vi "CSMclient.vi"(7 "CSM Name":string="CSM-Module") -> ()   [LabVIEW 2026, in "UI-距离测量.lvlib" / "UDP.lvlib"]
uses:
  UDP.lvlib
  Supports/UDP Settings.ctl
  Supports/UDP States.ctl
  <userlib>/_NEVSTOP/Communicable State Machine(CSM)/_Polymophic/CSM - Filter Duplicated Lines.vi
  93835eb5-cc1e-40fc-ad4c-6bcb3c5fabc0.vi
  <userlib>/_NEVSTOP/Communicable State Machine(CSM)/_Polymophic/CSM - Replace Marks in Messages.vi
  f33b5746-793c-4b4f-ac6a-ed109ca97768.vi
  <userlib>/_NEVSTOP/Communicable State Machine(CSM)/AdvanceAPI/CSM - Compact Multiple States.vi
  <userlib>/_NEVSTOP/Communicable State Machine(CSM)/AdvanceAPI/CSM - Break Down Multiple States String.vi
  <userlib>/_NEVSTOP/Communicable State Machine(CSM)/_Shared/Remove Comments from Single-line.vi
  <userlib>/_NEVSTOP/Communicable State Machine(CSM)/_Shared/Split Single-line Message.vi
  <userlib>/_NEVSTOP/Communicable State Machine(CSM)/_Shared/Trim Single-line Text.vi
  <userlib>/_NEVSTOP/Communicable State Machine(CSM)/AdvanceAPI/CSM - Revert Arguments-Safe String.vi
  <userlib>/_NEVSTOP/Communicable State Machine(CSM)/AdvanceAPI/CSM - Make String Arguments Safe.vi
  <userlib>/_NEVSTOP/Communicable State Machine(CSM)/AdvanceAPI/CSM - Keywords.vi
  <userlib>/_NEVSTOP/Communicable State Machine(CSM)/addons/API-String-Arugments-Support/_Support/Convert API String Arguments to Data(variant).vi
  <userlib>/_NEVSTOP/Communicable State Machine(CSM)/addons/API-String-Arugments-Support/_Support/Data To API String Arguments.vi
  <userlib>/_NEVSTOP/Communicable State Machine(CSM)/Communicable State Machine.lvlib
  <userlib>/_NEVSTOP/Communicable State Machine(CSM)/addons/Loop-Support/CSM Loop Support.lvlib
panel:
  in  "Start":bool
  in  "停止":bool
  out "data out":string
  out "Error Occurred":errorcluster
  out "State History":string
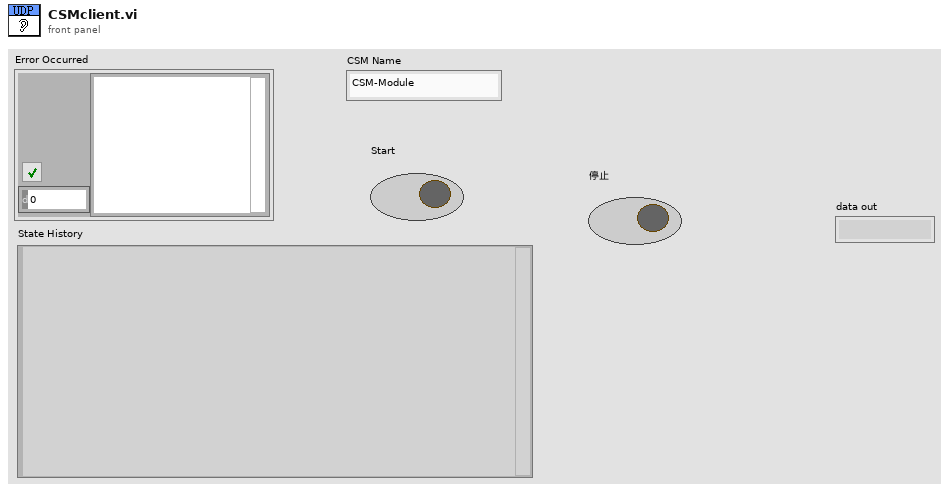
[diagram p1: front panel]
types:
  T1 = typedef "UI-距离测量.lvlib/UDP.lvlib/UDP Settings.ctl" = cluster{"连接ID":refnum<k16>, "网络地址(字符串)":string, "地址":u32, "本端口":u16, "对向":u16, "Read Interval":dbl, "Write Interval":dbl}
  T2 = enum32{"Invalid", "Standard", "Closed", "Hidden", "Minimized", "Maximized"}
  T3 = enum32{"invalid app kind", "Development System", "Run Time System", "Student Edition", "Embedded LabVIEW", "Evaluation", "Custom"}
  T4 = typedef "UI-距离测量.lvlib/UDP.lvlib/UDP States.ctl" = enum16{"Idle", "Acquiring", "Error"}
  T5 = typedef "Communicable State Machine.lvlib/_CSM_Response Source Message.ctl" = cluster{"‘State":string, "’Arguments":string, "’Error":errorcluster}
  T6 = cluster{"Current VI Reference":refnum<vi>, "Close Panel on Exit?":bool}
  T7 = cluster{"Core":cluster{"Current VI Reference":refnum<vi>, "Close Panel on Exit?":bool}, "State":T4, "UDP Settings":T1, "采集时间":timestamp}
  T8 = typedef "全局变量数据.ctl" = cluster{"温度采集":dbl[], "温度控制":dbl[], "压力测量":dbl[], "Zolix":dbl[], "步进电机":dbl[], "湿度测量":dbl[], "距离测量":dbl[]}
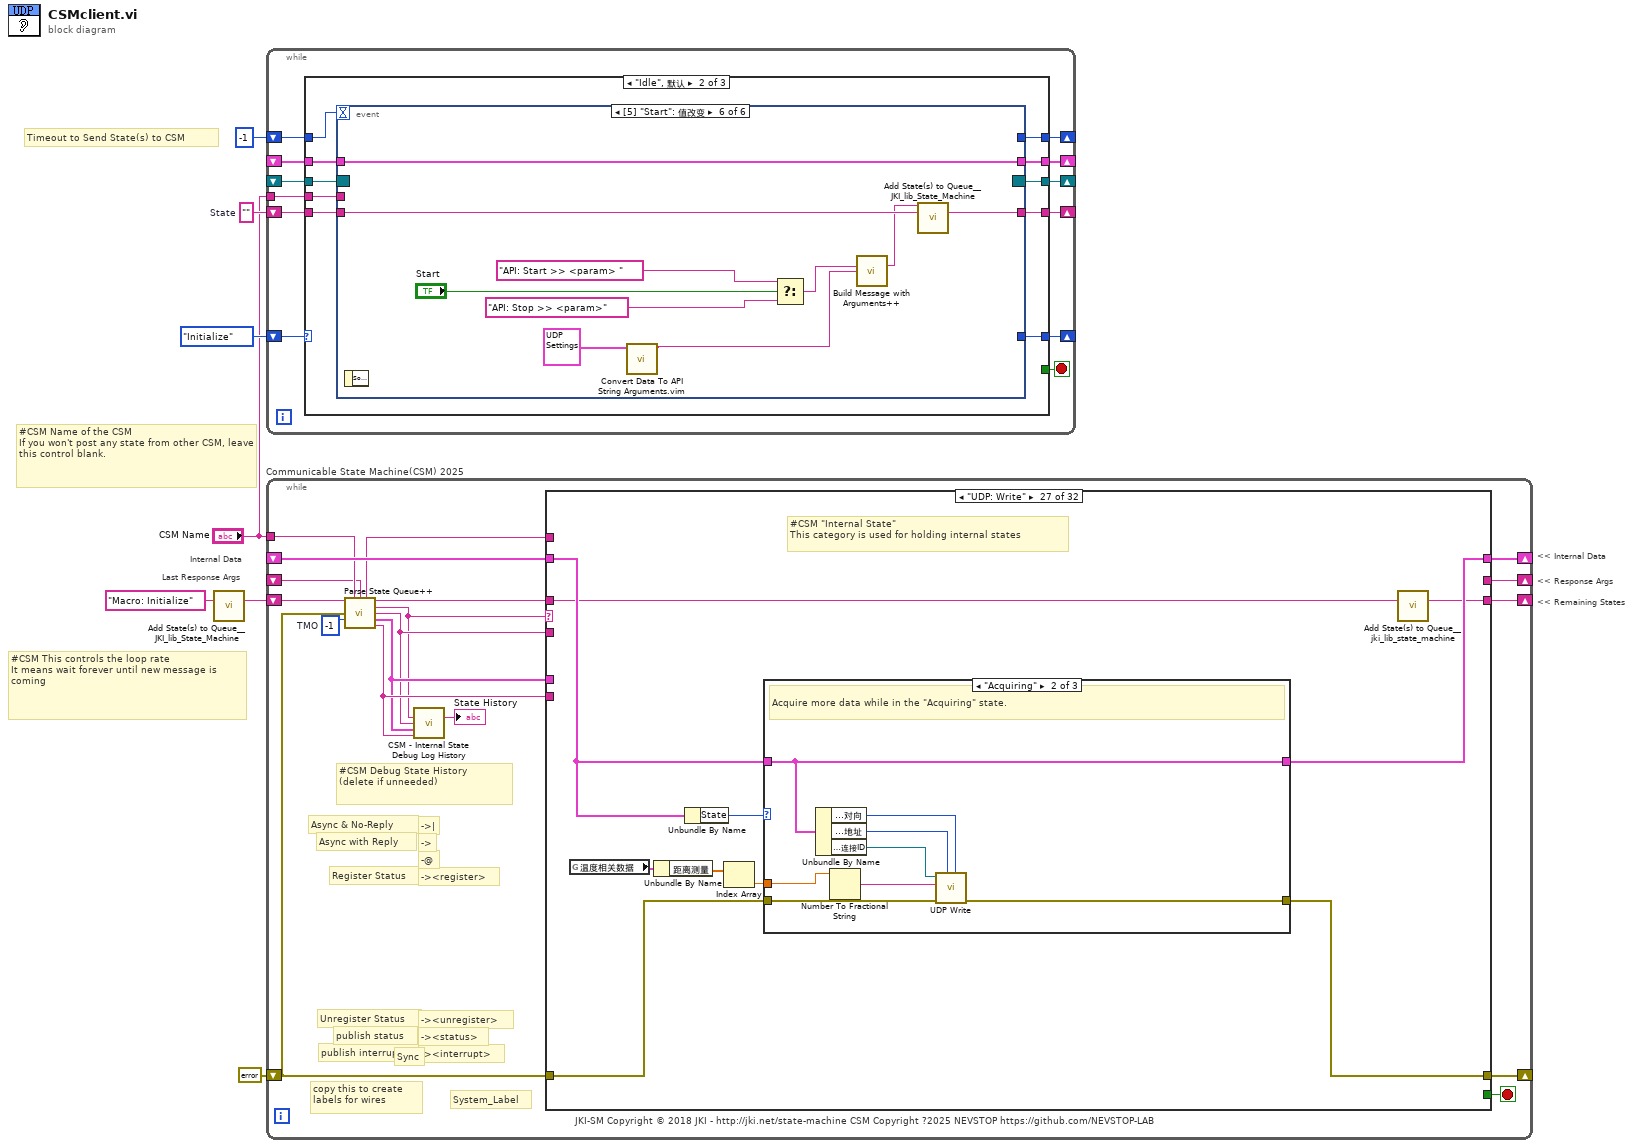
[diagram p0: block diagram]
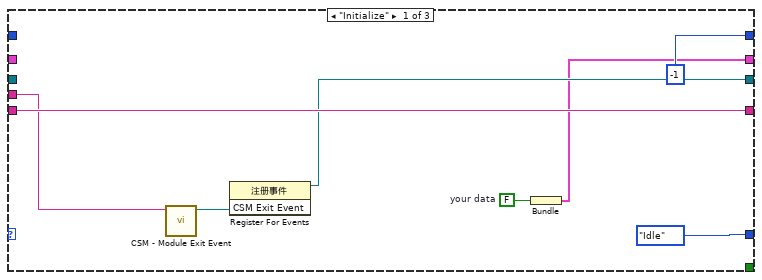
[diagram p2: hidden frame]
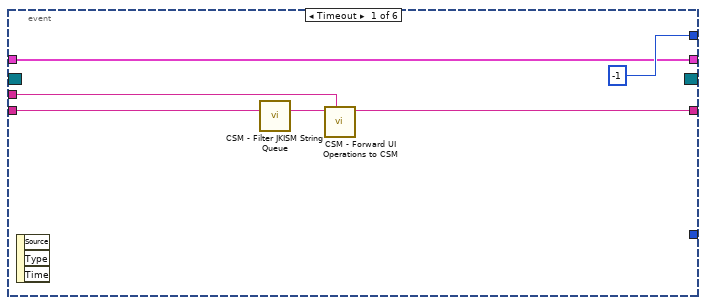
[diagram p3: hidden frame]
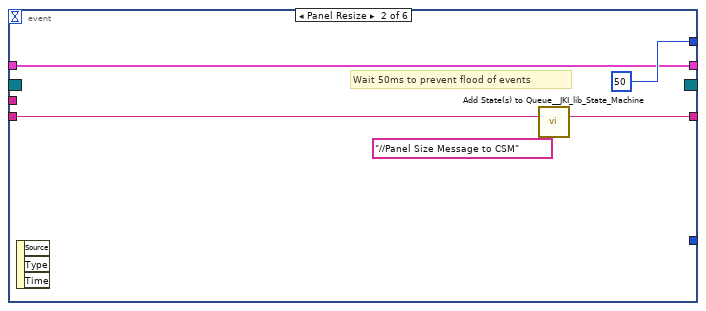
[diagram p4: hidden frame]
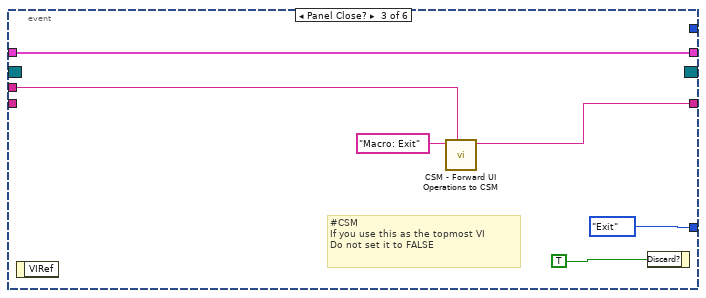
[diagram p5: hidden frame]
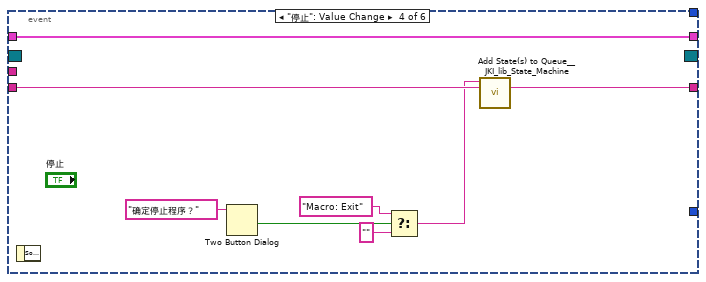
[diagram p6: hidden frame]
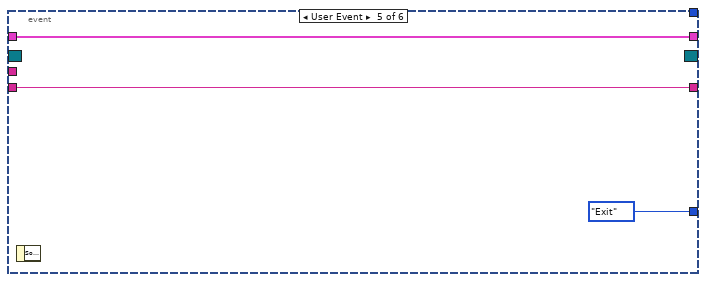
[diagram p7: hidden frame]
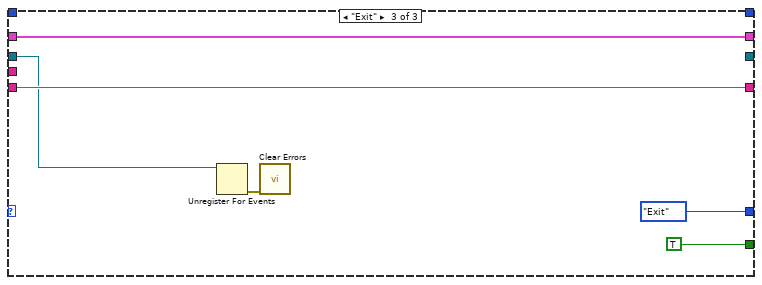
[diagram p8: hidden frame]
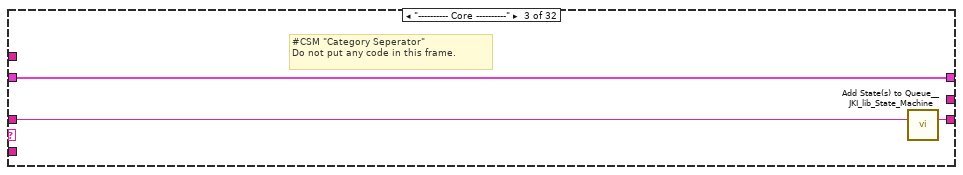
[diagram p11: hidden frame]
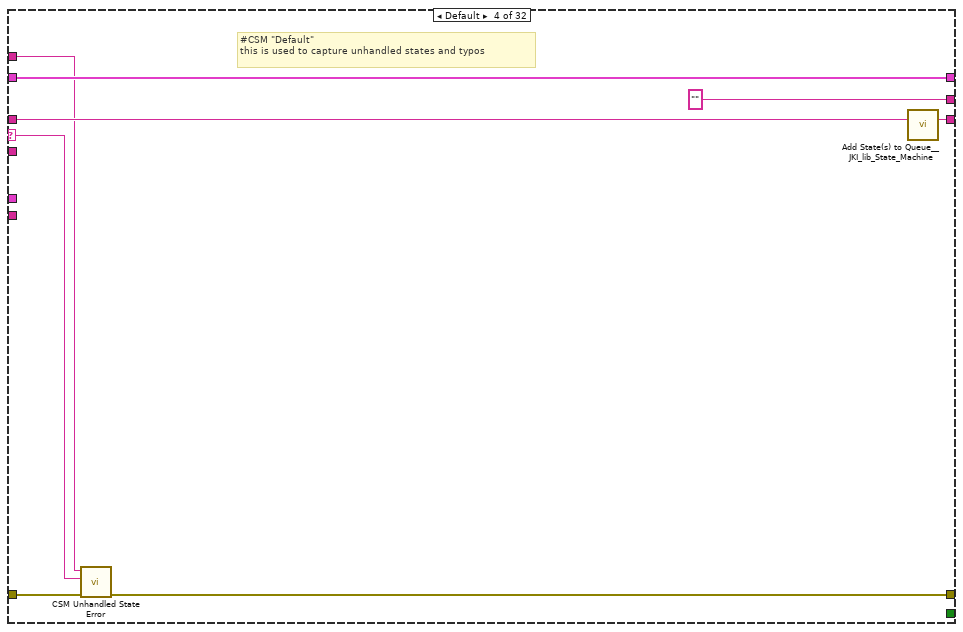
[diagram p12: hidden frame]
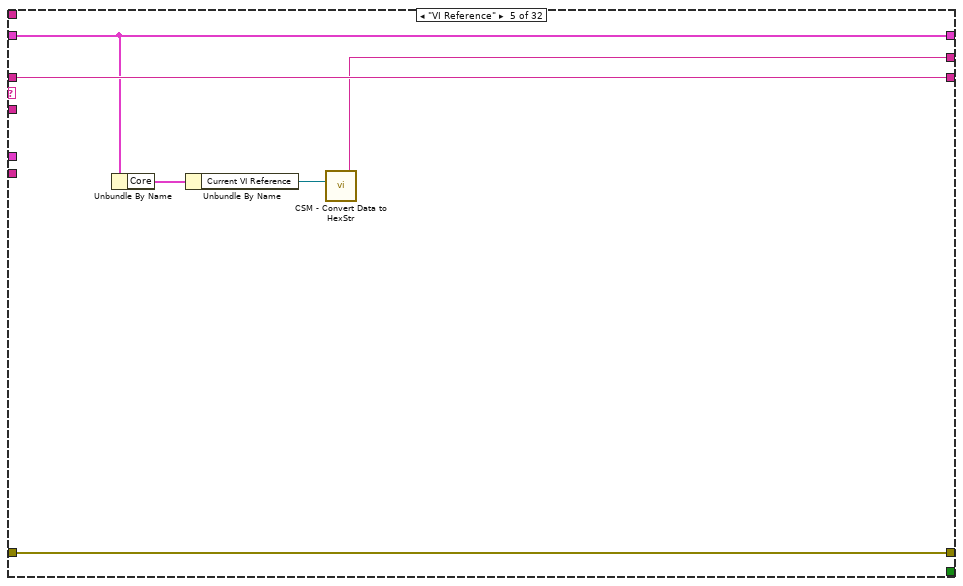
[diagram p13: hidden frame]
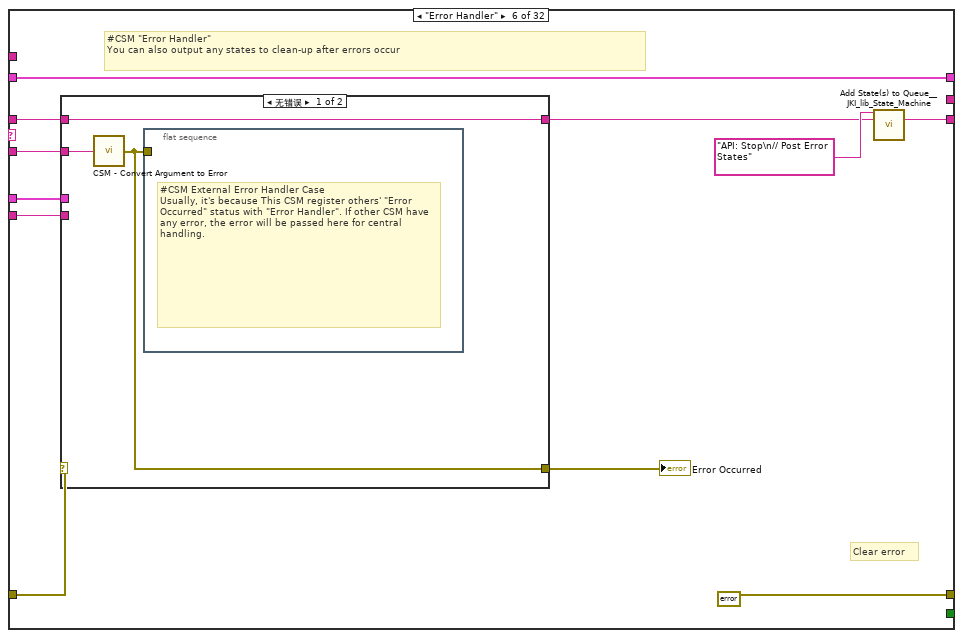
[diagram p14: hidden frame]
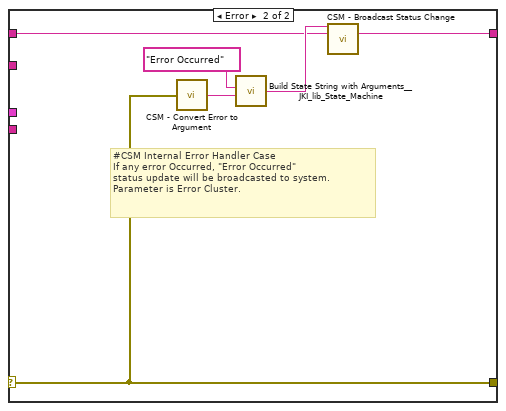
[diagram p15: hidden frame]
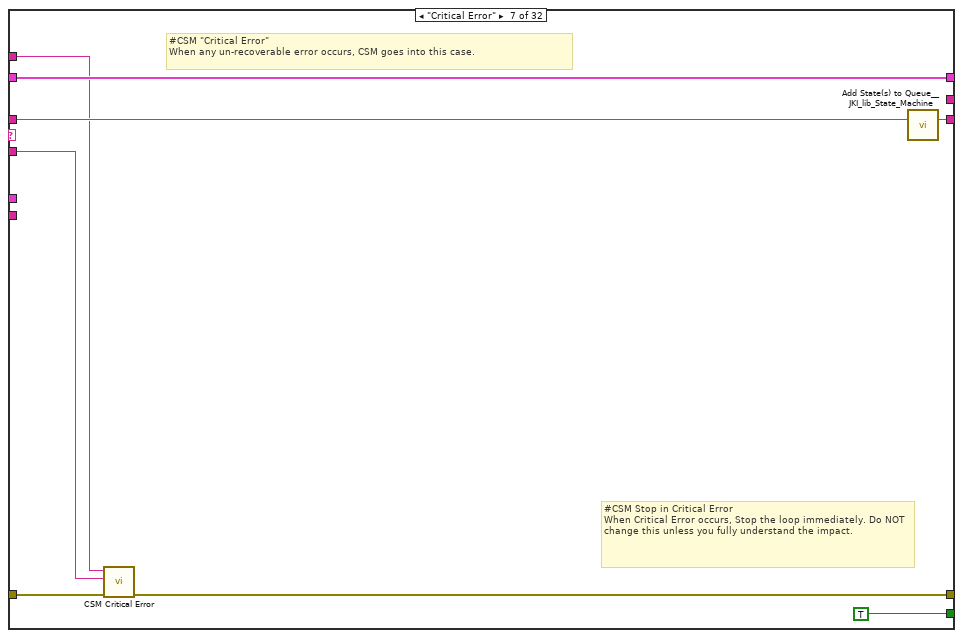
[diagram p16: hidden frame]
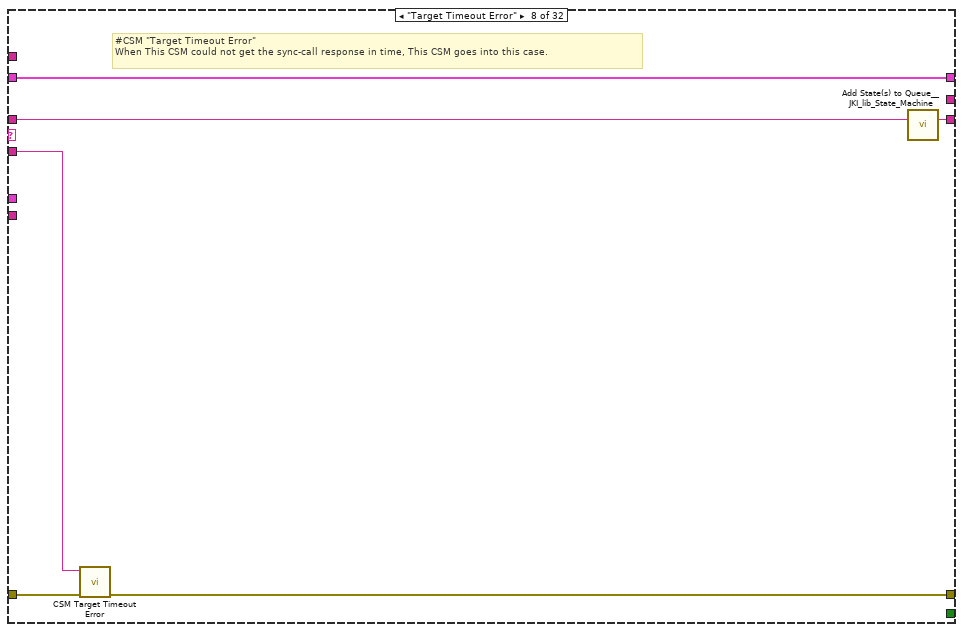
[diagram p17: hidden frame]
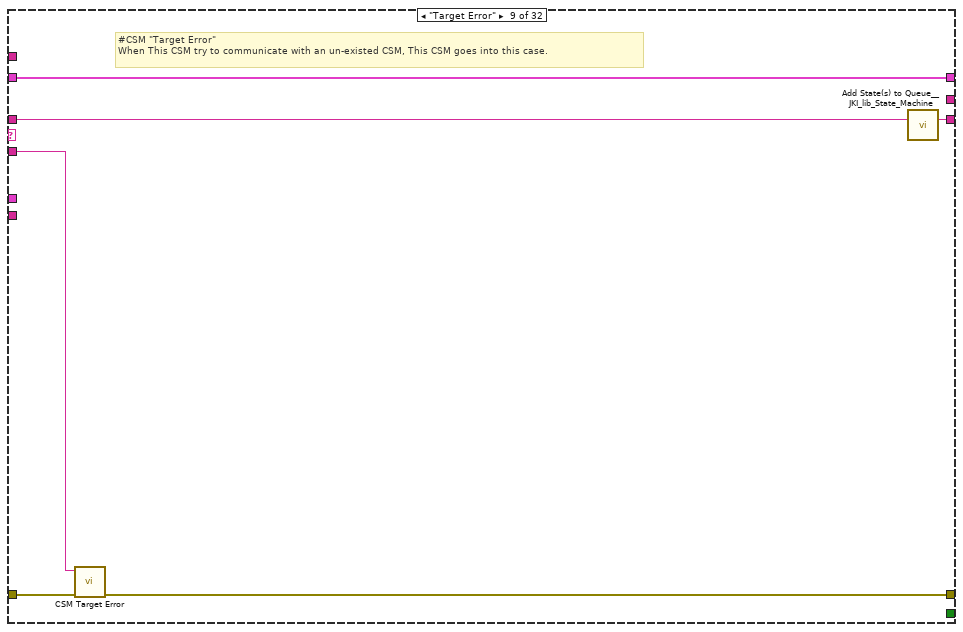
[diagram p18: hidden frame]
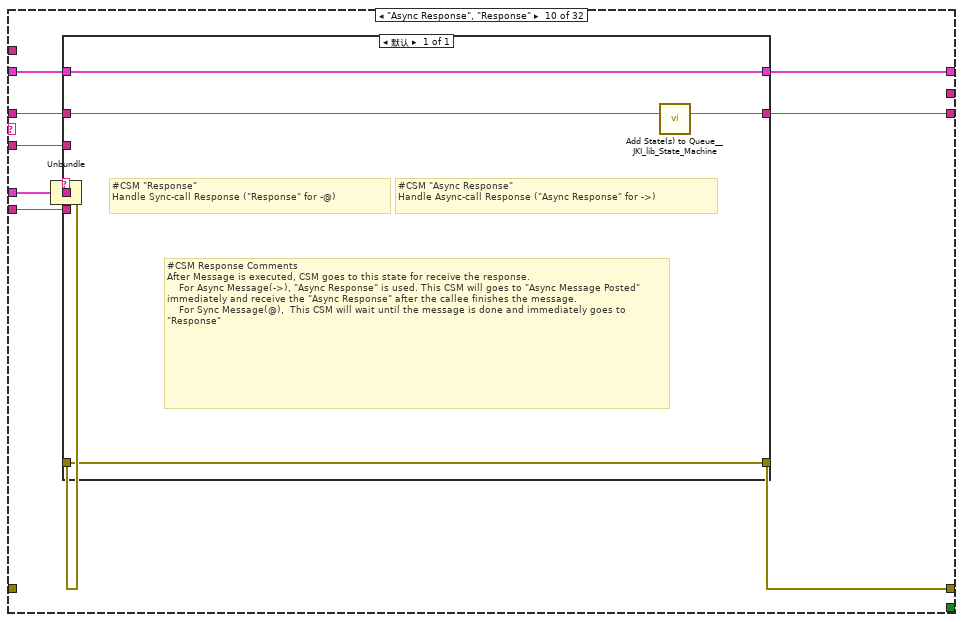
[diagram p19: hidden frame]
diagram:
  w3 = ""  # State
  # "Timeout to Send State(s) to CSM"
  # "Last Response Args"
  # "Internal Data"
  # "#CSM Name of the CSM\nIf you won't post any state from other CSM, leave this control blank."
  # "#CSM This controls the loop rate\nIt means wait forever until new message is coming"
  # "<< Internal Data"
  # "<< Response Args"
  # "<< Remaining States"
  n1 = call <vilib>:"Add State(s) to Queue__JKI_lib_State_Machine.vi"("State(s) in (\"\")"="Macro: Initialize" ("Init State(\"Macro: Initialize\")")) -> ("States Out"=w5:string)  [unwired: 14 in]
  n2 = while {
    shift-right: [w18] -> _
    shift-left: enum16{"Idle", "Initialize", "Exit"}."Initialize" -> [w19]
    tunnel: "CSM Name" -> [w16]
    shift-right: [w14] -> _
    shift-left: w3 -> [w15]
    shift-right: [w12] -> _
    shift-left: -1 -> [w13]
    shift-right: [w11] -> _
    shift-left: _ -> [w10]
    shift-right: [w9] -> _
    shift-left: _ -> [w8]
    stop <- w17 stop-if-true
    n3 = case shown="\"Idle\", 默认" w19 {
      tunnel: [enum16{"Idle", "Initialize", "Exit"}."Idle" w37 enum16{"Idle", "Initialize", "Exit"}."Exit"] -> w18
      tunnel: [_ _ TRUE] -> w17
      tunnel: w16 -> [w23 w36 _]
      tunnel: w15 -> [w26 w34 w79]
      tunnel: [w26 w35 w79] -> w14
      tunnel: w13 -> [_ w32 _]
      tunnel: [-1 w33 _] -> w12
      tunnel: [w22 w30 _] -> w11
      tunnel: w10 -> [_ w31 w78]
      tunnel: [w20 w28 w76] -> w9
      tunnel: w8 -> [_ w29 w76]
      frame "Initialize" {
        w21 = FALSE  # your data
        n4 = call <userlib>:"CSM - Module Exit Event.vi"("Name (\"\" to Use UUID) In"=w23) -> ("CSM Exit Event"=w24:refnum<user-event>)  [unwired: 8 in, 2 out]
        n5 = register-events(w24) -> (reference out=w22:refnum<event-registration>)  [unwired: 2 in, 1 out]
        n6 = Bundle("your data"=w21) -> (w20:cluster{"your data":bool})  [unwired: 1 in]
      }
      frame "Idle", Default {
        n7 = event shown="[5] \"Start\": 值改变" {
          selector: w31 -> [_ _ _ _ _ _]
          dyn-events: [_ _ _ _ _ _] -> w30
          timeout: w32 -> [_ _ _ _ _ _]
          tunnel: [_ _ enum16{"Idle", "Initialize", "Exit"}."Exit" _ enum16{"Idle", "Initialize", "Exit"}."Exit" _] -> w37
          tunnel: w36 -> [w39 _ w51 _ _ _]
          tunnel: w34 -> [w42 w48 _ w56 w65 w73]
          tunnel: [w40 w47 w50 w57 w65 w74] -> w35
          tunnel: [-1 50 _ _ _ _] -> w33
          tunnel: w29 -> [w38 w44 w49 w62 w63 w75]
          tunnel: [w38 w44 w49 w62 w63 w75] -> w28
          event Timeout {
            n8 = event-data() -> ()  [unwired: 1 in, 3 out]
            n9 = call-poly <userlib>:"CSM - Filter JKISM String Queue.vi"("States In"=w42) -> ("States Out"=w41:string)  [unwired: 14 in]
            n10 = call <userlib>:"CSM - Forward UI Operations to CSM.vi"("Name (\"\" to Use UUID)"=w39, "State(s) In (\"\")"=w41) -> ("States Out"=w40:string)  [unwired: 8 in, 1 out]
          }
          event Panel Resize {
            # "Wait 50ms to prevent flood of events"
            n11 = event-data() -> ()  [unwired: 1 in, 3 out]
            n12 = call <vilib>:"Add State(s) to Queue__JKI_lib_State_Machine.vi"("State(s) in (\"\")"=w48, "State(s) at Back (\"\")"="//Panel Size Message to CSM" ("State(s) at Back (\"\")")) -> ("States Out"=w47:string)  [unwired: 13 in]
          }
          event Panel Close? {
            # "#CSM \nIf you use this as the topmost VI\nDo not set it to FALSE"
            n13 = event-data() -> ()  [unwired: 1 in, 1 out]
            n14 = call <userlib>:"CSM - Forward UI Operations to CSM.vi"("Name (\"\" to Use UUID)"=w51, "State(s) In (\"\")"="Macro: Exit" ("State")) -> ("States Out"=w50:string)  [unwired: 8 in, 1 out]
            n15 = event-data("Discard?"=TRUE) -> ()  [unwired: 1 in, 1 out]
          }
          event "停止": Value Change {
            n16 = event-data() -> ()  [unwired: 1 in, 1 out]
            n17 = Two Button Dialog(message="确定停止程序？" ("消息")) -> (T button?=w61:bool)  [unwired: 2 in]
            n18 = Select(t="Macro: Exit" ("State(s) in Front (\"\")"), s=w61, f="") -> (s? t:f=w55:string)
            n19 = call <vilib>:"Add State(s) to Queue__JKI_lib_State_Machine.vi"("State(s) in Front (\"\")"=w55, "State(s) in (\"\")"=w56) -> ("States Out"=w57:string)  [unwired: 13 in]
          }
          event User Event {
            n20 = event-data() -> ()  [unwired: 1 in, 1 out]
          }
          event "Start": Value Change {
            n21 = event-data() -> ()  [unwired: 1 in, 1 out]
            n22 = call "Convert Data To API String Arguments.vim"("Data"=T1 {"连接ID"=refnum, "网络地址(字符串)"="", "地址"=0, "本端口"=12346, "对向"=12345, "Read Interval"=0.1, "Write Interval"=0.1} ("UDP Settings")) -> ("API String"=w72:string)  [unwired: 7 in, 1 out]
            n23 = Select(t="API: Start >> <param> " ("State"), s="Start", f="API: Stop >> <param>" ("State")) -> (s? t:f=w71:string)
            n24 = call-poly <userlib>:"Build Message with Arguments++.vi"("States With Replace Token"=w71, "<param>"=w72) -> ("States"=w67:string)  [unwired: 13 in]
            n25 = call <vilib>:"Add State(s) to Queue__JKI_lib_State_Machine.vi"("State(s) in Front (\"\")"=w67, "State(s) in (\"\")"=w73) -> ("States Out"=w74:string)  [unwired: 13 in]
          }
        }
      }
      frame "Exit" {
        n26 = Unregister For Events(event registration refnum=w78) -> (error out=w77:errorcluster)  [unwired: 1 in]
        n27 = call <vilib>:"Clear Errors.vi"("error in (no error)"=w77) -> ()  [unwired: 5 in, 2 out]
      }
    }
  }
  n28 = while "Communicable State Machine(CSM) 2025" {
    shift-right: [w94] -> _
    shift-left: _ -> [w93]
    shift-right: [w97] -> _
    shift-left: errorcluster {"status"=FALSE, "code"=0, "source"=""} ("error out") -> [w83]
    shift-right: [w96] -> _
    shift-left: w5 -> [w98]
    tunnel: "CSM Name" -> [w90]
    shift-right: [w91] -> _
    shift-left: _ -> [w85]
    stop <- w95 stop-if-true
    w92 = -1  # TMO
    # "#CSM Debug State History\n(delete if unneeded)"
    # "-><interrupt>"
    # "-><status>"
    # "-><unregister>"
    # "-><register>"
    # "-@"
    # "->"
    # "->|"
    # "publish interrupt"
    # "publish status"
    # "Unregister Status"
    # "Register Status"
    # "Sync"
    # "Async with Reply"
    # "Async & No-Reply"
    # "JKI-SM Copyright © 2018 JKI - http://jki.net/state-machine CSM Copyright ?2025 NEVSTOP https://github.com/NEVSTOP-LAB"
    # "copy this to create labels for wires"
    # "System_Label"
    n29 = call <userlib>:"Parse State Queue++.vi"("State Queue"=w98, "Name (\"\" to Use UUID)"=w90, "Response Arguments"=w85, "Previous Error"=w83, "Dequeue (1 ms)"=w92) -> ("Name Used"=w84:string, "Remaining States"=w99:string, "Current State"=w86:string, "Arguments"=w87:string, "Additional Information"=w88:T5, "Source CSM"=w89:string)  [unwired: 5 in]
    n30 = call <userlib>:"CSM - Internal State Debug Log History.vi"("State"=w86, "Arguments (\"\")"=w87, ">> Response Source Message >>"=w88, "Source (\"\")"=w89) -> ("Debug Log"=→"State History":string)  [unwired: 11 in]
    n31 = case shown="\"UDP: Write\"" w86 {
      selector: w86 -> [_ _ _ w110 _ _ _ _ _ _ _ _ _ _ _ _ _ _ _ _ _ _ _ _ _ _ _ _ _ _ w342 _]
      tunnel: w99 -> [w100 w103 w106 w114 w119 w125 w148 w154 w160 w170 w177 w189 w193 w196 w203 w207 w213 w216 w220 w228 w233 w243 w256 w263 w271 w273 w300 w321 w330 w333 w343 w348]
      tunnel: w87 -> [_ _ _ _ _ w124 w144 w151 w157 w164 _ _ _ _ _ _ _ _ _ _ _ w240 _ _ _ _ _ _ _ _ w340 _]
      tunnel: w93 -> [w101 w102 w104 w112 w118 w130 w146 w152 w158 w168 w176 w183 w191 w194 _ w206 w208 w214 w218 w224 w234 w236 w257 w261 w269 w275 w302 w319 w326 w331 w339 w347]
      tunnel: [_ _ _ w107 w120 errorcluster {"status"=FALSE, "code"=0, "source"=""} ("error out") w141 w149 w155 w171 _ _ _ _ _ _ w209 _ _ _ _ _ _ _ w268 w277 w304 _ _ _ _ w349] -> w97
      tunnel: w83 -> [_ _ _ w108 w120 w128 w142 w150 w156 _ _ _ _ _ _ _ w210 _ _ _ _ _ _ _ w268 w278 w305 _ w324 _ _ w349]
      tunnel: [w100 w103 w105 w113 w119 w126 w147 w153 w159 w169 w177 w188 w192 w195 w202 w207 w212 w215 w219 w227 w232 w242 w255 w262 w271 w274 w301 w320 w329 w332 w341 w346] -> w96
      tunnel: [_ _ _ _ _ _ TRUE _ _ _ _ _ TRUE _ _ _ _ _ _ _ _ _ _ _ _ _ _ _ _ _ _ _] -> w95
      tunnel: [w101 w102 w104 w112 w118 w130 w146 w152 w158 w167 w176 w187 w191 w194 w201 w206 w208 w214 w218 w224 w234 w235 w257 w261 w270 w276 w303 w319 w328 w331 w339 w347] -> w94
      tunnel: w89 -> [_ _ _ _ _ w123 _ _ _ w165 _ _ _ _ _ _ _ _ _ _ _ _ _ _ _ _ _ _ _ _ _ _]
      tunnel: w88 -> [_ _ _ _ _ w122 _ _ _ w166 _ _ _ _ _ _ _ _ _ _ _ _ _ _ _ _ _ _ _ _ _ _]
      tunnel: [_ _ _ "" w115 _ _ _ _ _ _ _ _ _ _ _ _ _ _ _ _ _ _ _ _ _ _ _ _ _ _ _] -> w91
      tunnel: w84 -> [_ _ _ w109 _ _ w143 _ _ _ _ _ _ _ _ _ _ _ _ _ _ _ _ _ _ _ _ _ _ _ _ _]
      frame "", "Idle" {
        # "#CSM \"Idle/Event Handler\"\nexecutes when the state queue is empty"
      }
      frame "CSM Documentation" {
        # "#CSM State Syntax\n\n// Comment line, all text to the right of “//” will be ignored\n// Local Message Example\nDoSth: DoA >> Arguments\n\n// Sync Call Example\nAPI: xxxx >> Arguments -@ TargetModule\n\n// Async Call Example\nAPI: xxxx >> Arguments -> TargetModule\n\n// Async Call without Reply Example\nAPI: xxxx >> Arguments ->| TargetModule\n\n// Broadcast normal status:\nStatus >> StatusArguments  -><status>\n\n// Broadcast Interrupt status:\nInterrupt >> StatusArguments  -><interrupt>\n\n// Register Source Module's status to Handler Module\nStatus@Source Module >> Handler Module@Handler Module -><register>\n\n// Unegister Source Module's status\nStatus@Source Module >> Handler Module -><unregister>"
        # "#CSM README FIRST\n\nCommunicable State Machine(CSM) is a LabVIEW application framework that builds upon JKI State Machine(JKISM). It follows the pattern of JKISM and extends the keywords to describe message communication between modules, including concepts such as Sync-Message, Async-Message, Subscription/Unsubscription of status - essential elements for creating reusable code modules. For more information, please visit the CSM wiki: https://nevstop-lab.github.io/CSM-Wiki/\n\nFor instructions on JKI State Machine, visit: \n    http://jki.net/state-machine/\nFor information about CSM, visit: \n    https://github.com/NEVSTOP-LAB"
        # "#CSM \"Documentation\"\nCase for holding CSM Documenation"
      }
      frame "---------- Core ----------" {
        # "#CSM \"Category Seperator\"\nDo not put any code in this frame."
        n32 = call <vilib>:"Add State(s) to Queue__JKI_lib_State_Machine.vi"("State(s) in (\"\")"=w106) -> ("States Out"=w105:string)  [unwired: 14 in]
      }
      frame Default {
        # "#CSM \"Default\"\nthis is used to capture unhandled states and typos"
        n33 = call <userlib>:"CSM Unhandled State Error.vi"("error in (no error)"=w108, "Undefined State"=w110, "CSM Name"=w109) -> ("error out"=w107:errorcluster)  [unwired: 8 in]
        n34 = call <vilib>:"Add State(s) to Queue__JKI_lib_State_Machine.vi"("State(s) in (\"\")"=w114) -> ("States Out"=w113:string)  [unwired: 14 in]
      }
      frame "VI Reference" {
        n35 = Unbundle By Name(w118) -> ("Core"=w117:T6)
        n36 = Unbundle By Name(w117) -> ("Current VI Reference"=w116:refnum<vi>)
        n37 = call <userlib>:"CSM - Convert Data to HexStr.vi"("Variant"=w116) -> ("HEX String (0-9,A-F)"=w115:string)  [unwired: 8 in]
      }
      frame "Error Handler" {
        # "#CSM \"Error Handler\"\nYou can also output any states to clean-up after errors occur"
        # "Clear error"
        n38 = case shown="无错误" w128 {
          selector: w128 -> [_ w135]
          tunnel: [w134 w137] -> w127
          tunnel: w125 -> [w134 w136]
          tunnel: w124 -> [w133 _]
          tunnel: w123 -> [_ _]
          tunnel: w122 -> [_ _]
          tunnel: [w132 w135] -> w121
          frame No Error {
            n39 = call <userlib>:"CSM - Convert Argument to Error.vi"("Argument"=w133) -> ("Error"=w132:errorcluster)  [unwired: 4 in]
            n40 = flat-sequence {
              tunnel: w132 -> [_]
              frame #0 {
                # "#CSM External Error Handler Case\nUsually, it's because This CSM register others' \"Error Occurred\" status with \"Error Handler\". If other CSM have any error, the error will be passed here for central handling."
              }
            }
          }
          frame Error {
            # "#CSM Internal Error Handler Case \nIf any error Occurred, \"Error Occurred\" \nstatus update will be broadcasted to system.\nParameter is Error Cluster."
            n41 = call <userlib>:"CSM - Convert Error to Argument.vi"("Error"=w135) -> ("Argument"=w139:string)  [unwired: 4 in]
            n42 = call <vilib>:"Build State String with Arguments__JKI_lib_State_Machine.vi"("Arguments (\"\")"=w139, "State"="Error Occurred" ("Status with Arguments")) -> ("State with Arguments"=w138:string)  [unwired: 4 in]
            n43 = call <userlib>:"CSM - Broadcast Status Change.vi"("Status With Arguments"=w138, "State Queue"=w136) -> ("Remaining States"=w137:string)  [unwired: 13 in]
          }
        }
        "Error Occurred" <- w121
        n44 = call <vilib>:"Add State(s) to Queue__JKI_lib_State_Machine.vi"("State(s) in Front (\"\")"="API: Stop\n// Post Error States", "State(s) in (\"\")"=w127) -> ("States Out"=w126:string)  [unwired: 13 in]
      }
      frame "Critical Error" {
        # "#CSM \"Critical Error\"\nWhen any un-recoverable error occurs, CSM goes into this case."
        # "#CSM Stop in Critical Error\nWhen Critical Error occurs, Stop the loop immediately. Do NOT change this unless you fully understand the impact."
        n45 = call <userlib>:"CSM Critical Error.vi"("error in (no error)"=w142, "Arugments (As Reason)"=w144, "CSM Name"=w143) -> ("error out"=w141:errorcluster)  [unwired: 8 in]
        n46 = call <vilib>:"Add State(s) to Queue__JKI_lib_State_Machine.vi"("State(s) in (\"\")"=w148) -> ("States Out"=w147:string)  [unwired: 14 in]
      }
      frame "Target Timeout Error" {
        # "#CSM \"Target Timeout Error\"\nWhen This CSM could not get the sync-call response in time, This CSM goes into this case."
        n47 = call <userlib>:"CSM Target Timeout Error.vi"("error in (no error)"=w150, "Arguments (As CSM Name)"=w151) -> ("error out"=w149:errorcluster)  [unwired: 9 in]
        n48 = call <vilib>:"Add State(s) to Queue__JKI_lib_State_Machine.vi"("State(s) in (\"\")"=w154) -> ("States Out"=w153:string)  [unwired: 14 in]
      }
      frame "Target Error" {
        # "#CSM \"Target Error\"\nWhen This CSM try to communicate with an un-existed CSM, This CSM goes into this case."
        n49 = call <userlib>:"CSM Target Error.vi"("error in (no error)"=w156, "Arguments (As CSM Name)"=w157) -> ("error out"=w155:errorcluster)  [unwired: 9 in]
        n50 = call <vilib>:"Add State(s) to Queue__JKI_lib_State_Machine.vi"("State(s) in (\"\")"=w160) -> ("States Out"=w159:string)  [unwired: 14 in]
      }
      frame "Async Response", "Response" {
        n51 = Unbundle(w166) -> ("‘State"=w163:string, "’Arguments"=w162:string, "’Error"=w161:errorcluster)
        n52 = case shown="默认" w163 {
          tunnel: [w172] -> w169
          tunnel: w170 -> [w173]
          tunnel: [w175] -> w167
          tunnel: w168 -> [w175]
          tunnel: [w174] -> w171
          tunnel: w161 -> [w174]
          tunnel: w165 -> [_]
          tunnel: w164 -> [_]
          tunnel: w162 -> [_]
          frame 默认 {
            # "#CSM \"Async Response\"\nHandle Async-call Response (\"Async Response\" for ->)"
            # "#CSM \"Response\"\nHandle Sync-call Response (\"Response\" for -@)"
            # "#CSM Response Comments\nAfter Message is executed, CSM goes to this state for receive the response.\n    For Async Message(->), \"Async Response\" is used. This CSM will goes to \"Async Message Posted\" immediately and receive the \"Async Response\" after the callee finishes the message.\n    For Sync Message(@),  This CSM will wait until the message is done and immediately goes to \"Response\""
            n53 = call <vilib>:"Add State(s) to Queue__JKI_lib_State_Machine.vi"("State(s) in (\"\")"=w173) -> ("States Out"=w172:string)  [unwired: 14 in]
          }
        }
      }
      frame "Async Message Posted" {
        # "#CSM \"Async Message Posted\"\nAfter Async Message is posted (-> or ->| ), CSM goes to this state for post-action.\nYou can use Argument - State to tell which Async Message is called."
      }
      frame "Initialize Core Data" {
        # "#CSM \"Initialize Core Data\"\nThis is used to determine panel behavior on exit"
        # "originally closed?"
        # "exe?"
        # "If panel starts closed or is an EXE, then close it when we exit"
        n54 = property class="VI"() -> ("FP.State"=w180:T2)  [unwired: 2 in, 2 out]
        n55 = property class="App"() -> ("App.Kind"=w186:T3)  [unwired: 2 in, 2 out]
        n56 = control-ref of="Current VI Reference"() -> (w181:refnum<vi>)
        n57 = Equal?(x=w180, y=T2."Closed" ("Front Panel Window:State")) -> (x = y?=w178:bool)
        n58 = Equal?(x=w186, y=T3."Run Time System" ("Application:Kind")) -> (x = y?=w184:bool)
        n59 = Or(x=w178, y=w184) -> (x .or. y?=w182:bool)
        n60 = Bundle By Name(cluster=w183, "Core.Current VI Reference"=w181, "Core.Close Panel on Exit?"=w182) -> (w187:T7)
        n61 = call <vilib>:"Add State(s) to Queue__JKI_lib_State_Machine.vi"("State(s) in (\"\")"=w189) -> ("States Out"=w188:string)  [unwired: 14 in]
      }
      frame "Exit" {
        # "#CSM \"Exit\"\nCase for exiting the loop. No errors that occur here will be handled."
        n62 = call <vilib>:"Add State(s) to Queue__JKI_lib_State_Machine.vi"("State(s) in (\"\")"=w193) -> ("States Out"=w192:string)  [unwired: 14 in]
      }
      frame "---------- Data ----------" {
        # "#CSM \"Category Seperator\"\nDo not put any code in this frame."
        n63 = call <vilib>:"Add State(s) to Queue__JKI_lib_State_Machine.vi"("State(s) in (\"\")"=w196) -> ("States Out"=w195:string)  [unwired: 14 in]
      }
      frame "Data: Initialize" {
        w197 = T1 {"连接ID"=refnum, "网络地址(字符串)"="", "地址"=0, "本端口"=12346, "对向"=12345, "Read Interval"=0.1, "Write Interval"=0.1}  # UDP Settings
        w198 = timestamp(0 s since 1904-01-01)  # 采集时间
        w199 = UDP_States."Idle"  # State
        w200 = T6 {"Current VI Reference"=refnum, "Close Panel on Exit?"=FALSE}  # Core
        # "#CSM \"Data: Initialize\"\nInitialize the shift-register data, here.\n(data names are defined by what you wire into the bundle function)"
        # "#CSM do not delete - used by framework"
        # "#CSM Data names and types of shift register data are defined by this bundle."
        n64 = Bundle("Core"=w200, "State"=w199, "UDP Settings"=w197, "采集时间"=w198) -> (w201:T7)  [unwired: 1 in]
        n65 = call <vilib>:"Add State(s) to Queue__JKI_lib_State_Machine.vi"("State(s) in (\"\")"=w203) -> ("States Out"=w202:string)  [unwired: 14 in]
      }
      frame "Data: Update Indicators" {
        n66 = local write "Start"(FALSE ("Start")) -> ()
        n67 = local write "Error Occurred"(errorcluster {"status"=FALSE, "code"=0, "source"=""} ("错误常量")) -> ()
      }
      frame "Data: Cleanup" {
        # "#CSM \"Data: Cleanup\"\nCleanup any data and references, here.\n(this is called automatically, by the Macro: Exit)"
        n68 = Unbundle By Name(w208) -> ("Core.Current VI Reference"=w211:refnum<vi>)
        n69 = Close Reference(reference=w211, error in (no error)=w210) -> (error out=w209:errorcluster)
        n70 = call <vilib>:"Add State(s) to Queue__JKI_lib_State_Machine.vi"("State(s) in (\"\")"=w213) -> ("States Out"=w212:string)  [unwired: 14 in]
      }
      frame "---------- Macro ----------" {
        # "#CSM \"Category Seperator\"\nDo not put any code in this frame."
        n71 = call <vilib>:"Add State(s) to Queue__JKI_lib_State_Machine.vi"("State(s) in (\"\")"=w216) -> ("States Out"=w215:string)  [unwired: 14 in]
      }
      frame "Macro: Initialize" {
        # "#CSM \"Macro: Initialize\"\nInitialization Macro (This is called once, when the VI starts)"
        n72 = call <vilib>:"Add State(s) to Queue__JKI_lib_State_Machine.vi"("State(s) in Front (\"\")"="Data: Initialize\nInitialize Core Data\nData: Update Indicators", "State(s) in (\"\")"=w220) -> ("States Out"=w219:string)  [unwired: 13 in]
      }
      frame "Macro: Exit" {
        # "#CSM \"Macro: Exit\"\nExit Macro (This is called once, when the VI exits)"
        n73 = Unbundle By Name(w224) -> ("State"=w223:T4)
        n74 = case shown="\"Acquiring\"" w223 {
          tunnel: ["" "Break Continuous\nUDP: Close" ""] -> w221
          frame "Idle", Default {
          }
          frame "Acquiring" {
          }
          frame "Error" {
          }
        }
        n75 = call <vilib>:"Add State(s) to Queue__JKI_lib_State_Machine.vi"("State(s) in Front (\"\")"="//Exit Sub-Modules ", "State(s) in (\"\")"=w221, "State(s) at Back (\"\")"="Data: Cleanup\nExit") -> ("States Out"=w225:string)  [unwired: 12 in]
        n76 = call <vilib>:"Add State(s) to Queue__JKI_lib_State_Machine.vi"("State(s) in Front (\"\")"=w225, "State(s) in (\"\")"=w228) -> ("States Out"=w227:string)  [unwired: 13 in]
      }
      frame "---------- API ----------" {
        # "#CSM \"Category Seperator\"\nDo not put any code in this frame."
        n77 = call <vilib>:"Add State(s) to Queue__JKI_lib_State_Machine.vi"("State(s) in (\"\")"=w233) -> ("States Out"=w232:string)  [unwired: 14 in]
      }
      frame "API: Start" {
        w238 = T1 {"连接ID"=refnum, "网络地址(字符串)"="localhost", "地址"=0, "本端口"=12346, "对向"=12346, "Read Interval"=0.0, "Write Interval"=0.0}  # UDP Settings
        # "#CSM API Example\nCopy/Rename this case for your own API"
        n78 = Unbundle By Name(w236) -> ("State"=w245:T4)
        n79 = case shown="\"Idle\"" w245 {
          selector: w245 -> [_ w251 w252]
          tunnel: [UDP_States."Acquiring" ("Acquisition State") w251 w252] -> w246
          tunnel: ["UDP: Initialize \nUDP: Read\nContinuous Check >> UDP: Read -><loop> \nUDP: Stop\nUDP: Close" ("State(s) in Front (\"\")") _ _] -> w244
          frame "Idle" {
            # "If the system is idle, start the acquisition."
          }
          frame "Acquiring" {
            # "The system is already acquiring. Ignore the \"Start\" message."
          }
          frame "Error" {
          }
        }
        n80 = local write "Start"(TRUE ("Start")) -> ()
        n81 = local write "Error Occurred"(errorcluster {"status"=FALSE, "code"=0, "source"=""} ("错误常量")) -> ()
        n82 = call "Convert API String Arguments to Data.vim"("Reference Type"=w238, "API String"=w240) -> ("Data"=w239:T1)  [unwired: 6 in, 1 out]
        n83 = call <userlib>:"CSMLS - Define Loop State(s).vi"("Loop States"=w244, "States Queue"=w243) -> ("Remaining States"=w242:string)  [unwired: 13 in]
        n84 = in-place {
          in-place-border: w246 -> [w248]
          in-place-border: w239 -> [w247]
          n85 = in-place-cluster #1(w236) -> ()  [unwired: 2 out]
          n86 = in-place-cluster #1("State"=w248, "UDP Settings"=w247) -> (w235:T7)
        }
      }
      frame "API: Stop" {
        # "#CSM API Example\nCopy/Rename this case for your own API"
        n87 = Unbundle By Name(w257) -> ("State"=w258:T4)
        n88 = case shown="\"Acquiring\"" w258 {
          tunnel: [_ "Break Continuous" ("State(s) in Front (\"\")") "Break Continuous" ("State(s) in Front (\"\")")] -> w254
          frame "Idle" {
            # "The system is already idle. Ignore the \"Stop\" message."
          }
          frame "Acquiring" {
            # "If the system is acquiring, stop the acquisition."
          }
          frame "Error" {
          }
        }
        n89 = local write "Start"(FALSE ("Start")) -> ()
        n90 = call <vilib>:"Add State(s) to Queue__JKI_lib_State_Machine.vi"("State(s) in Front (\"\")"=w254, "State(s) in (\"\")"=w256) -> ("States Out"=w255:string)  [unwired: 13 in]
      }
      frame "---------- UDP ----------" {
        # "#CSM \"Category Seperator\"\nDo not put any code in this frame."
        n91 = call <vilib>:"Add State(s) to Queue__JKI_lib_State_Machine.vi"("State(s) in (\"\")"=w263) -> ("States Out"=w262:string)  [unwired: 14 in]
      }
      frame "UDP: Initialize" {
        # "#CSM \"Category Seperator\"\nDo not put any code in this frame."
        n92 = Unbundle By Name(w269) -> ("UDP Settings.网络地址(字符串)"=w264:string, "UDP Settings.本端口"=w266:u16)
        n93 = String To IP(1:w264) -> (0:w265:u32)
        n94 = UDP Open(11:w266) -> (port=w267:refnum<k16>)  [unwired: 4 in, 2 out]
        n95 = Bundle By Name(cluster=w269, "UDP Settings.地址"=w265, "UDP Settings.连接ID"=w267) -> (w270:T7)
      }
      frame "UDP: Read" {
        # "#CSM \"Internal State\"\nThis category is used for holding internal states"
        n96 = Unbundle By Name(w275) -> ("State"=w279:T4)
        n97 = case shown="\"Acquiring\"" w279 {
          selector: w279 -> [_ w283 _]
          tunnel: [w281 w290 w296] -> w277
          tunnel: w278 -> [w281 w291 w296]
          tunnel: [w280 w284 w295] -> w276
          tunnel: w275 -> [w280 w285 w295]
          frame "Idle" {
            # "Ignore \"Acquire\" messages when the acquisition is idle."
          }
          frame "Acquiring" {
            # "Acquire more data while in the \"Acquiring\" state."
            n98 = Unbundle By Name(w285) -> ("UDP Settings.连接ID"=w292:refnum<k16>)
            n99 = call "UDP Read.vi"("错误输入（无错误）"=w291, "连接ID"=w292) -> ("无错误"=w290:errorcluster, "data out"=w289:string)  [unwired: 7 in, 1 out]
            "data out" <- w289
            n100 = Get Date/Time In Seconds() -> (seconds since 1Jan1904=w282:timestamp)
            n101 = in-place {
              in-place-border: w283 -> [w294]
              in-place-border: w282 -> [w293]
              n102 = in-place-cluster #2(w285) -> ()  [unwired: 2 out]
              n103 = in-place-cluster #2("State"=w294, "采集时间"=w293) -> (w284:T7)
            }
            n104 = call <userlib>:"CSM - Run Script.vi"("CSM Scripts"=w289, "Continue If Error? (F)"=TRUE, "Wait (5000ms)"=200) -> ("error out"=w286:errorcluster)  [unwired: 10 in, 2 out]
            n105 = call <vilib>:"Clear Errors.vi"("error in (no error)"=w286) -> ()  [unwired: 5 in, 2 out]
          }
          frame "Error" {
          }
        }
        n106 = call <vilib>:"Add State(s) to Queue__jki_lib_state_machine.vi"("State(s) in Front (\"\")"="UDP: Write" ("State(s) in Front (\"\")"), "State(s) in (\"\")"=w273) -> ("States Out"=w274:string)  [unwired: 13 in]
      }
      frame "UDP: Write" {
        # "#CSM \"Internal State\"\nThis category is used for holding internal states"
        n107 = global read "辅助系统全局变量 - T1.vi" "温度相关数据"() -> (w299:T8)
        n108 = Unbundle By Name(w299) -> ("距离测量"=w298:dbl[])
        n109 = Unbundle By Name(w302) -> ("State"=w306:T4)
        n110 = Index Array(array=w298) -> (element=w297:dbl)  [unwired: 1 in]
        n111 = case shown="\"Acquiring\"" w306 {
          tunnel: [w308 w312 w318] -> w304
          tunnel: w305 -> [w308 w313 w318]
          tunnel: [w307 w309 w317] -> w303
          tunnel: w302 -> [w307 w309 w317]
          tunnel: w297 -> [_ w311 _]
          frame "Idle" {
            # "Ignore \"Acquire\" messages when the acquisition is idle."
          }
          frame "Acquiring" {
            # "Acquire more data while in the \"Acquiring\" state."
            n112 = Unbundle By Name(w309) -> ("UDP Settings.对向"=w315:u16, "UDP Settings.地址"=w314:u32, "UDP Settings.连接ID"=w316:refnum<k16>)
            n113 = Number To Fractional String(number=w311) -> (F-format string=w310:string)  [unwired: 3 in]
            n114 = call "UDP Write.vi"("对方端口"=w315, "地址"=w314, "错误输入（无错误）"=w313, "数据输入"=w310, "连接ID"=w316) -> ("错误输出"=w312:errorcluster)  [unwired: 5 in, 1 out]
          }
          frame "Error" {
          }
        }
        n115 = call <vilib>:"Add State(s) to Queue__jki_lib_state_machine.vi"("State(s) in (\"\")"=w300) -> ("States Out"=w301:string)  [unwired: 14 in]
      }
      frame "UDP: Stop" {
        # "#CSM \"Internal State\"\nThis category is used for holding internal states"
        n116 = call <vilib>:"Add State(s) to Queue__JKI_lib_State_Machine.vi"("State(s) in (\"\")"=w321) -> ("States Out"=w320:string)  [unwired: 14 in]
      }
      frame "UDP: Close" {
        w327 = UDP_States."Idle"  # State
        # "#CSM \"Internal State\"\nThis category is used for holding internal states"
        n117 = Unbundle By Name(w326) -> ("UDP Settings.连接ID"=w325:refnum<k16>)
        n118 = UDP Close(connection ID=w325, 8:w324) -> (error out=w323:errorcluster)  [unwired: 1 out]
        n119 = call <vilib>:"Clear Errors.vi"("error in (no error)"=w323) -> ()  [unwired: 5 in, 2 out]
        n120 = local write "Start"(FALSE ("Start")) -> ()
        n121 = Bundle By Name(cluster=w326, "State"=w327) -> (w328:T7)
        n122 = call <vilib>:"Add State(s) to Queue__JKI_lib_State_Machine.vi"("State(s) in (\"\")"=w330) -> ("States Out"=w329:string)  [unwired: 14 in]
      }
      frame "---------- Loop ----------" {
        # "#CSM \"Internal State\"\nThis category is used for holding internal states"
        n123 = call <vilib>:"Add State(s) to Queue__JKI_lib_State_Machine.vi"("State(s) in (\"\")"=w333) -> ("States Out"=w332:string)  [unwired: 14 in]
      }
      frame "Continuous Check" {
        # "#CSM \"Internal State\"\nThis category is used for holding internal states"
        n124 = Unbundle By Name(w339) -> ("UDP Settings.Read Interval"=w345:dbl, "采集时间"=w337:timestamp)
        n125 = Get Date/Time In Seconds() -> (seconds since 1Jan1904=w338:timestamp)
        n126 = Multiply(x=u32 1000 ("y"), y=w345) -> (x*y=w336:dbl)
        n127 = Subtract(x=w338, y=w337) -> (x-y=w335:dbl)
        n128 = Subtract(x=w336, y=w335) -> (x-y=w334:dbl)
        n129 = Wait (ms)(milliseconds to wait=w334) -> ()  [unwired: 1 out]
        n130 = call <userlib>:"CSMLS - Append Continuous State.vi"("Loop State(s) And Arguments"=w340, "Continous Arguments (\"\")"=w340, "Continous State"=w342, "States Queue"=w343) -> ("Remaining States"=w341:string)  [unwired: 7 in]
      }
      frame "Break Continuous" {
        n131 = call <userlib>:"CSMLS - Remove Loop Tag to Break.vi"("States Queue"=w348) -> ("Remaining States"=w346:string)  [unwired: 10 in]
      }
    }
  }
